vi "Frame_Pace.vi"(0 "Start ms":u32, 1 "Count":i32, 11 "error in":errorcluster) -> (4 "Start out":u32, 6 "Count out":i32, 15 "error out":errorcluster)   [LabVIEW 2020, in "GH_App.lvlib"]
doc: "Paces the game loop at exactly 60 ticks per second (the screen refresh rate): waits until Start + (Count + 1) * 1000 / 60 ms. Count <= 0 starts the clock now; more than 50 ms behind (a hitch) restarts it, so the game never races to catch up."
uses:
  GH_App.lvlib
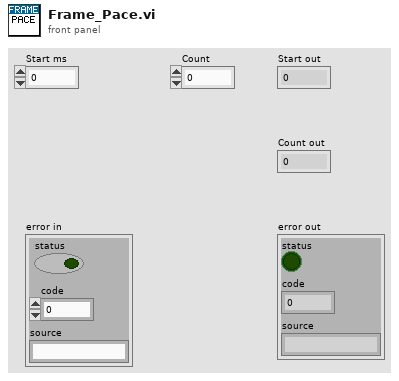
[diagram p1: front panel]
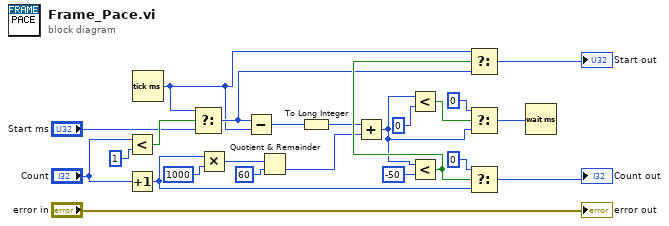
[diagram p0: block diagram]
diagram:
  n1 = Less?(x="Count", y=1) -> (x < y?=w6:bool)
  n2 = Increment(x="Count") -> (x+1=w8:i32)
  n3 = Tick Count (ms)() -> (millisecond timer value=w4:u32)
  n4 = Select(t=w4, s=w6, f="Start ms") -> (s? t:f=w7:u32)
  n5 = Multiply(x=w8, y=1000) -> (x*y=w10:i32)
  n6 = Subtract(x=w7, y=w4) -> (x-y=w13:u32)
  n7 = Quotient & Remainder(x=w10, y=60) -> (floor(x/y)=w12:i32)  [unwired: 1 out]
  n8 = To Long Integer(number=w13) -> (32bit integer=w14:i32)
  n9 = Add(x=w14, y=w12) -> (x+y=w15:i32)
  n10 = Less?(x=w15, y=0) -> (x < y?=w19:bool)
  n11 = Less?(x=w15, y=-50) -> (x < y?=w17:bool)
  n12 = Select(t=w4, s=w17, f=w7) -> (s? t:f=→"Start out":u32)
  n13 = Select(t=0, s=w19, f=w15) -> (s? t:f=w21:i32)
  n14 = Select(t=0, s=w17, f=w8) -> (s? t:f=→"Count out":i32)
  n15 = Wait (ms)(milliseconds to wait=w21) -> ()  [unwired: 1 out]
  "error out" <- "error in"
